vi "Preallocate-Reentrant.vi"   [LabVIEW 2023]
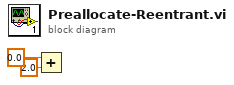
[diagram p0: block diagram]
diagram:
  n1 = Add(x=0.0, y=2.0) -> ()  [unwired: 1 out]
